vi "Array Panel Async.vi"(8 "ExecAnchor":refnum<class "ExecAnchor.lvclass">, 10 "Container":refnum<vi>, 11 "PanelArray in":refnum<class "ArrayManager.lvclass">) -> ()   [LabVIEW 2020, in "OOPanel.lvlib" / "ArrayManager.lvclass"]
uses:
  ArrayManager.lvclass
  lv-exec-anchor/ExecAnchor/ExecAnchor.lvclass
  UI State.ctl
  Events.ctl
  Scroll Into View.ctl
  ArrayManager.lvclass/ArrayManager.ctl
  ArrayPanel/ArrayPanel.lvclass
  C:/dev/lv20CE/relink/lv-oopanel/OOPanel/Panel/Panel.lvclass
  Panel/Panel.lvclass
panel:
  out "Page Size":dbl
  in  "Scrollbar":i32(c297)
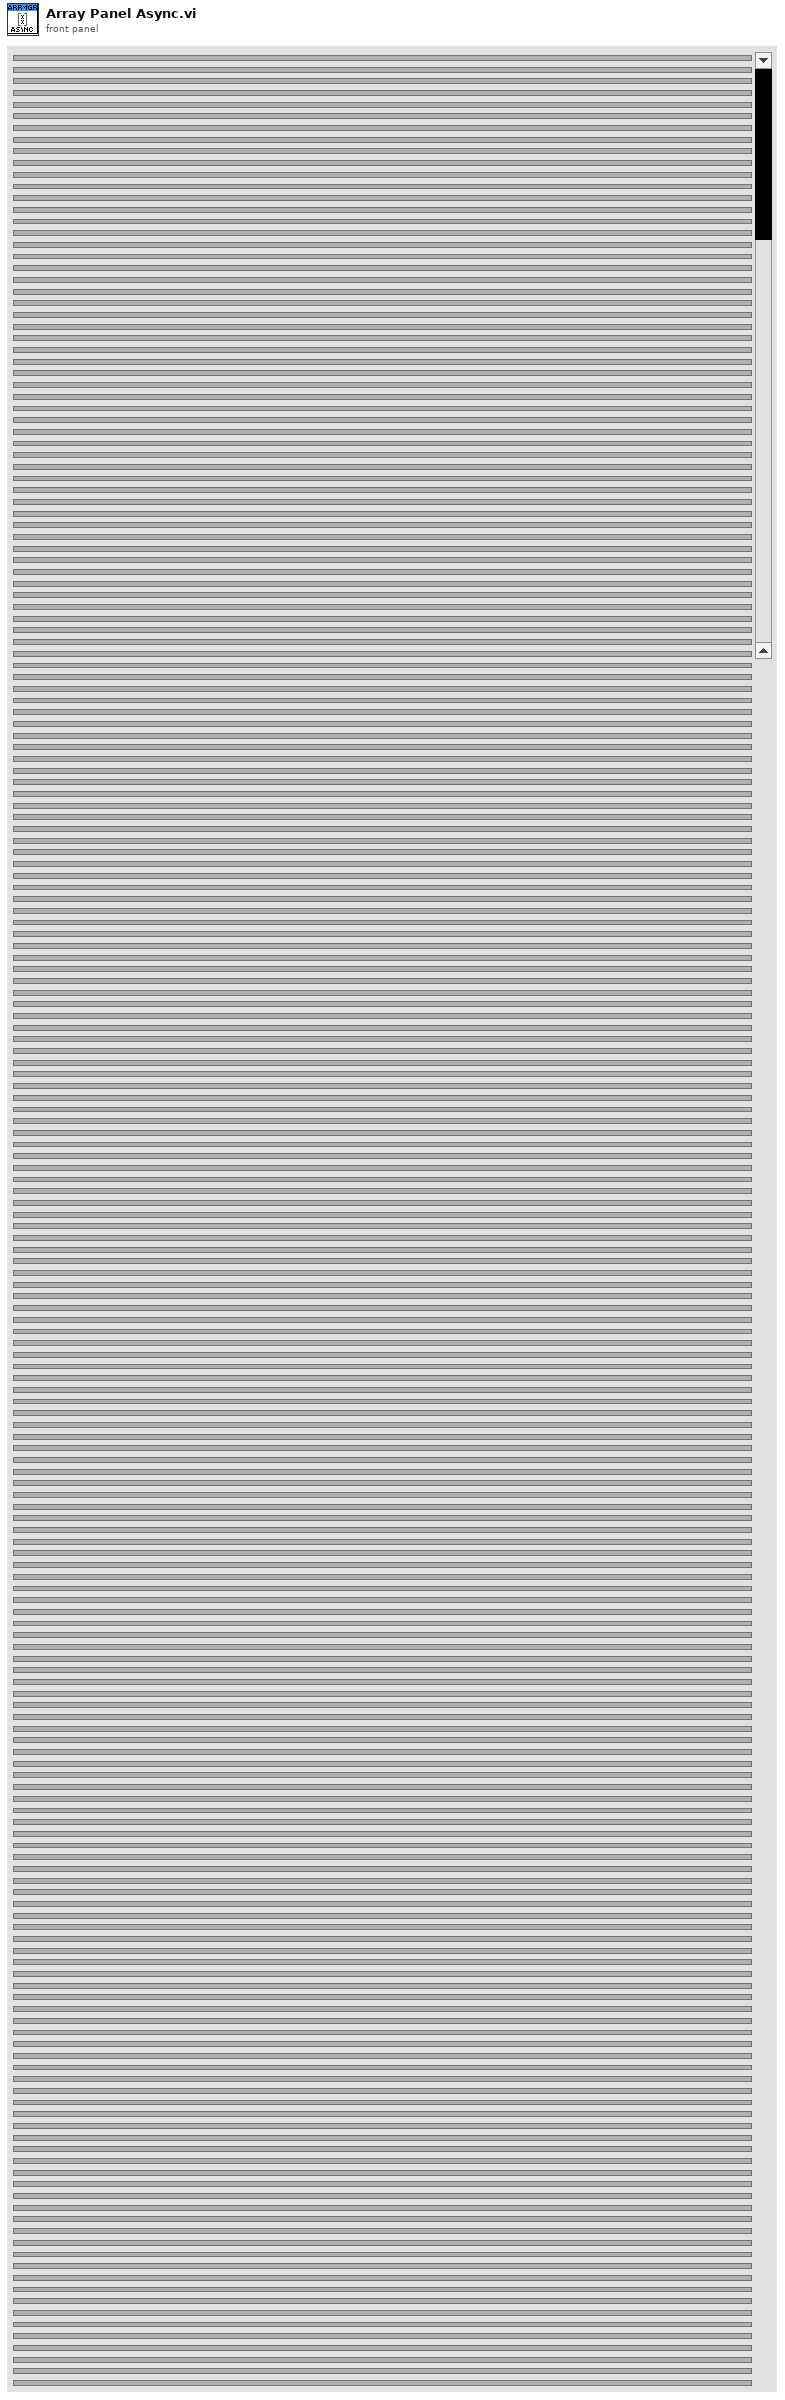
[diagram p1: front panel]
types:
  T1 = typedef "OOPanel.lvlib/ArrayManager.lvclass/UI State.ctl" = enum16{"Init", "Run", "Close"}
  T2 = cluster{"Panel":refnum<event-registration>, "ExecAnchor":refnum<event-registration>}
  T3 = typedef "OOPanel.lvlib/ArrayManager.lvclass/State Ref.ctl" = cluster{"Running":bool, "Borders":bool, "Total Height":dbl, "Scroll Visible":bool, "Background":u32}
  T4 = typedef "OOPanel.lvlib/ArrayManager.lvclass/UI Refs.ctl" = cluster{"SubPanels":refnum<vi>[], "Scrollbar":refnum<vi>, "Panel VI":refnum<vi>, "Container":refnum<vi>}
  T5 = typedef "OOPanel.lvlib/ArrayManager.lvclass/Events.ctl" = cluster{"Stop":refnum<user-event>, "Update":refnum<user-event>, "Scroll":refnum<user-event>, "Set BG":refnum<user-event>, "Scroll To Panel":refnum<user-event>, "Highlight":refnum<user-event>}
  T6 = typedef "OOPanel.lvlib/Desired Size.ctl" = cluster{"Width":u32, "Height":u32}
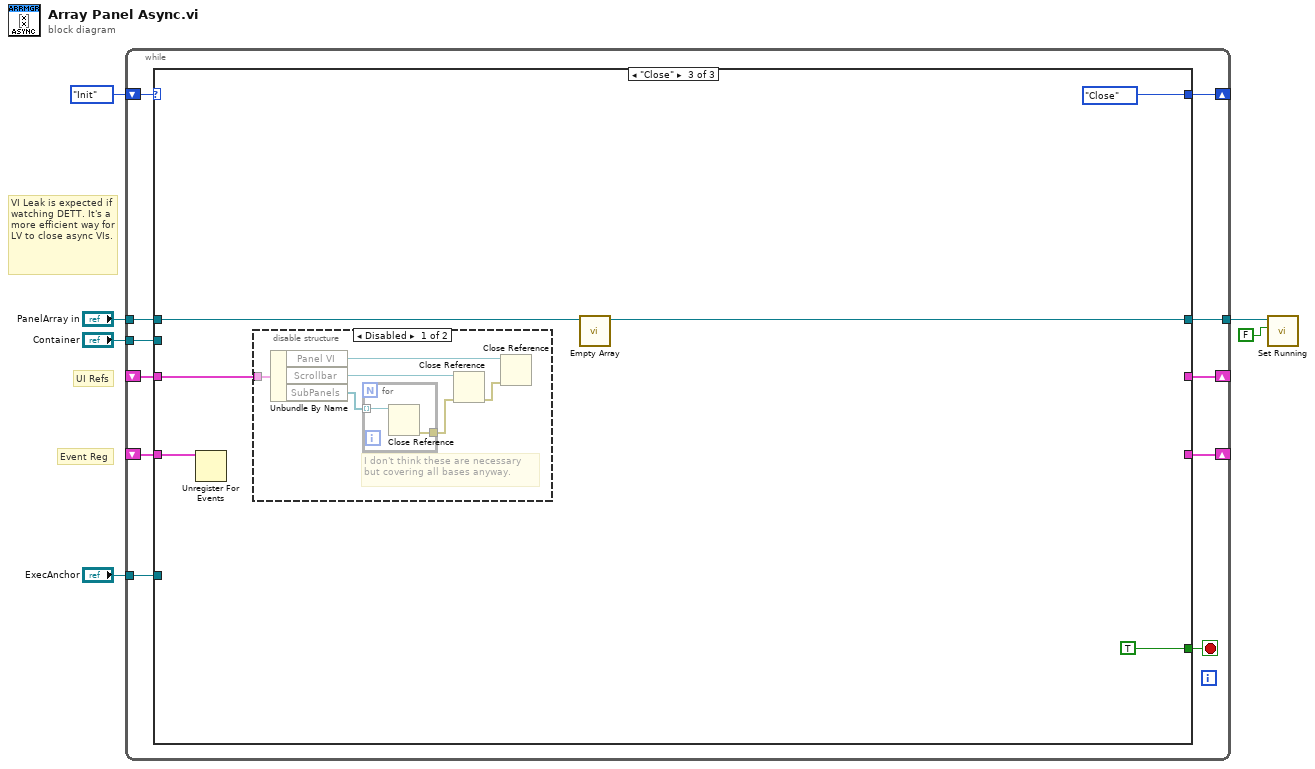
[diagram p0: block diagram]
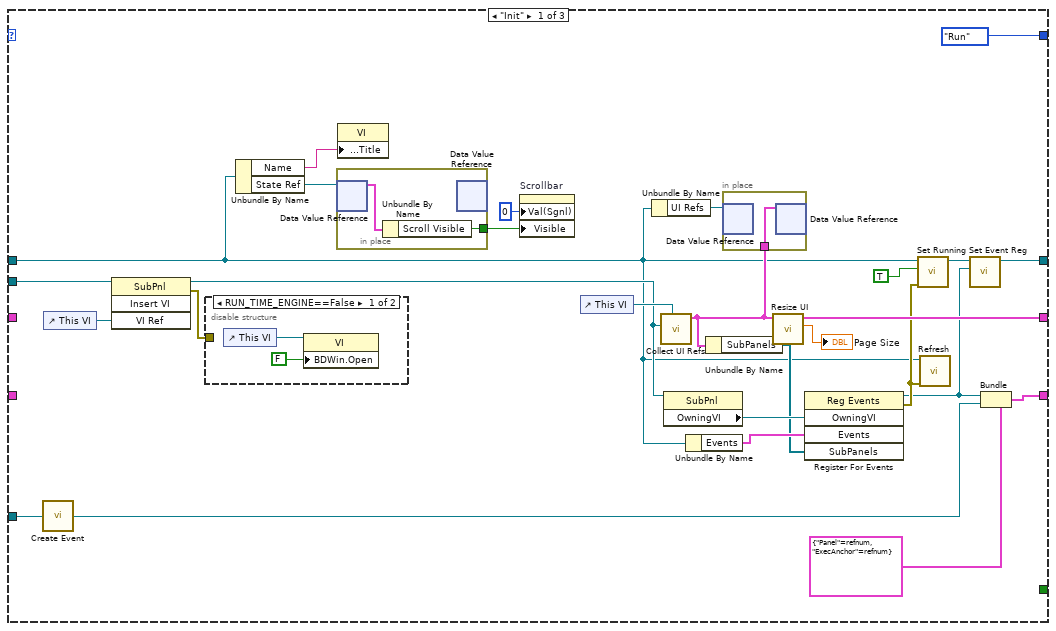
[diagram p2: hidden frame]
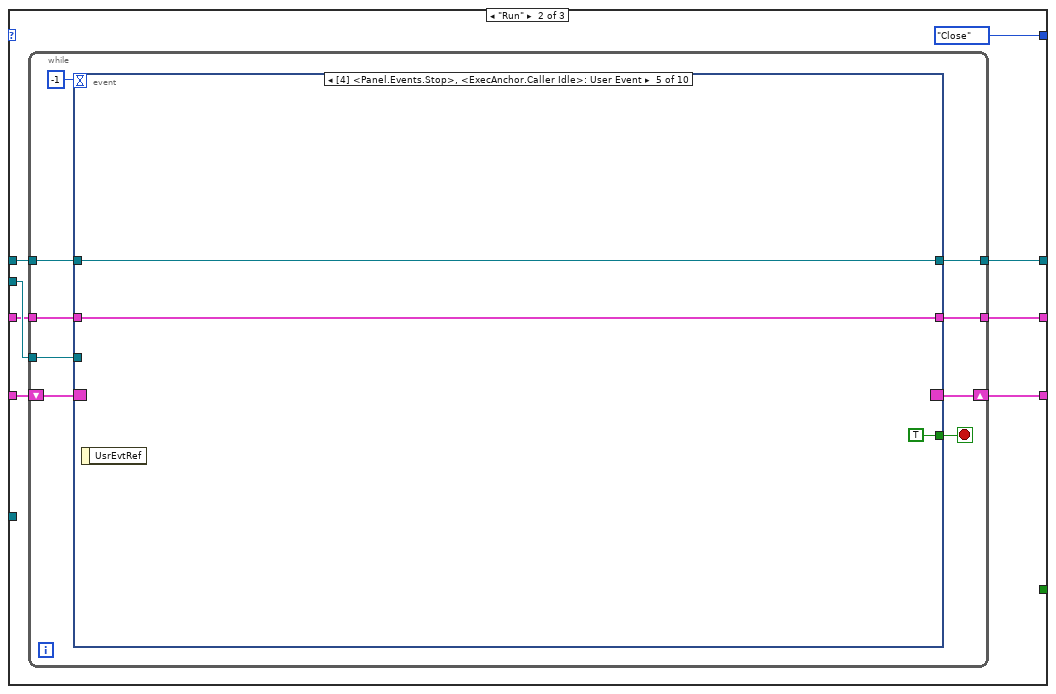
[diagram p4: hidden frame]
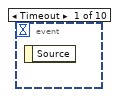
[diagram p5: hidden frame]
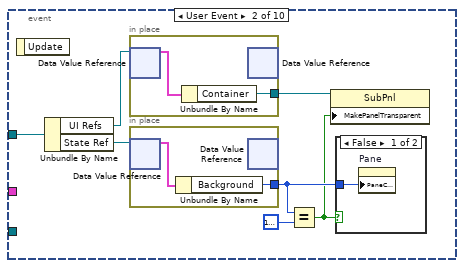
[diagram p6: hidden frame]
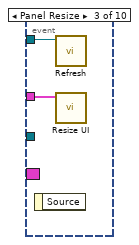
[diagram p8: hidden frame]
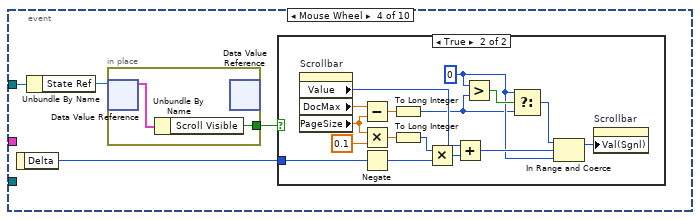
[diagram p9: hidden frame]
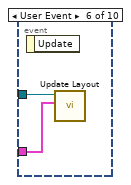
[diagram p11: hidden frame]
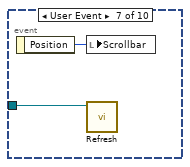
[diagram p12: hidden frame]
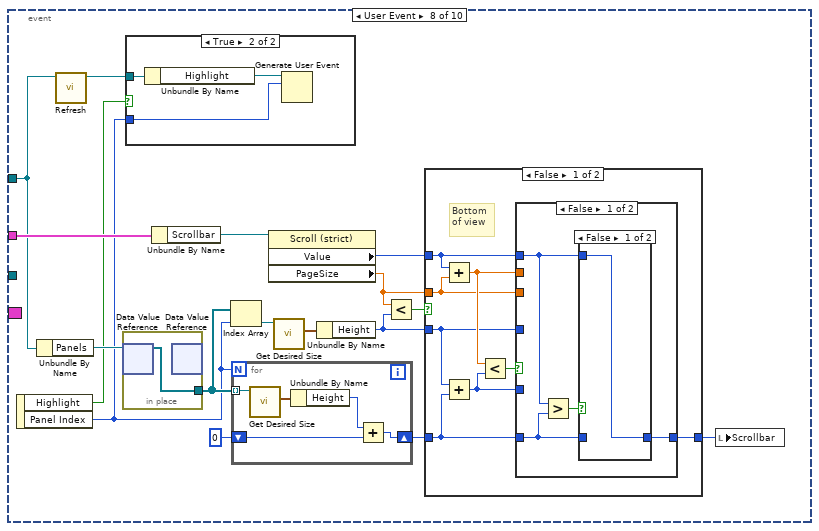
[diagram p13: hidden frame]
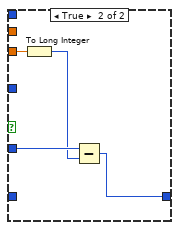
[diagram p16: hidden frame]
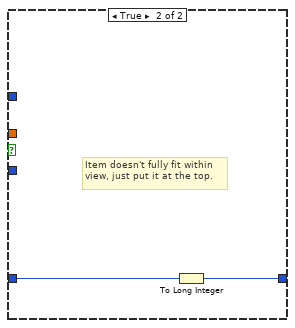
[diagram p17: hidden frame]
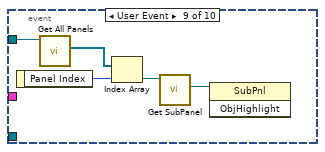
[diagram p18: hidden frame]
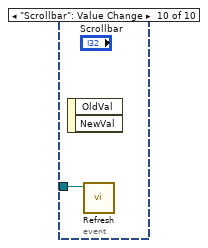
[diagram p19: hidden frame]
diagram:
  # "VI Leak is expected if watching DETT. It's a more efficient way for LV to close async VIs."
  # "Event Reg"
  # "UI Refs"
  n1 = while {
    shift-right: [w16] -> _
    shift-left: UI_State."Init" ("UI State") -> [w17]
    tunnel: "PanelArray in" -> [w15]
    tunnel: "Container" -> [w13]
    shift-right: [w12] -> _
    shift-left: _ -> [w11]
    shift-right: [w10] -> _
    shift-left: _ -> [w9]
    tunnel: [w8] -> w4
    tunnel: "ExecAnchor" -> [w7]
    stop <- w14 stop-if-true
    n2 = case shown="\"Close\"" w17 {
      tunnel: [UI_State."Run" ("UI State") UI_State."Close" ("UI State") UI_State."Close" ("UI State")] -> w16
      tunnel: w15 -> [w22 w56 w163]
      tunnel: [_ _ TRUE] -> w14
      tunnel: w13 -> [w37 w55 _]
      tunnel: [w18 w54 _] -> w12
      tunnel: w11 -> [_ w53 w165]
      tunnel: [w40 w51 _] -> w10
      tunnel: w9 -> [_ w52 w164]
      tunnel: [w25 w50 w162] -> w8
      tunnel: w7 -> [w21 _ _]
      frame "Init" {
        n3 = call "Create Event.vi"("ExecAnchor in"=w21) -> ("Event Reg"=w20:refnum<event-registration>)  [unwired: 3 in, 1 out]
        n4 = control-ref of="This VI"() -> (w36:refnum<vi>)
        n5 = invoke class="SubPnl" method="Insert VI"(reference=w37, "VI Ref"=w36) -> (reference out=w35:refnum<vi>, error out=w34:errorcluster)  [unwired: 2 in, 2 out]
        n6 = disable-structure shown="RUN_TIME_ENGINE==False" {
          disable-tunnel: w34 -> [_ _]
          frame condition #0 (active) {
            n7 = control-ref of="This VI"() -> (w49:refnum<vi>)
            n8 = property class="VI"(reference=w49, "BDWin.Open"=FALSE ("Block Diagram Window:Open")) -> ()  [unwired: 1 in, 2 out]
          }
          frame condition #1 {
          }
        }
        n9 = Unbundle By Name(w22) -> ("Name"=w23:string, "State Ref"=w31:refnum<data-value>)
        n10 = in-place {
          in-place-border: [w46] -> w30
          n11 = in-place-dvr #1(w31) -> (w47:T3)  [unwired: 1 out]
          n12 = Unbundle By Name(w47) -> ("Scroll Visible"=w46:bool)
          n13 = in-place-dvr #1() -> ()  [unwired: 1 in, 2 out]
        }
        n14 = property class="VI"("Front Panel.Title"=w23) -> ()  [unwired: 2 in, 2 out]
        n15 = property on="Scrollbar" class="Scroll (strict)"("Val(Sgnl)"=0 ("Value (Signaling)"), "Visible"=w30) -> ()  [unwired: 2 in, 2 out]
        n16 = control-ref of="This VI"() -> (w43:refnum<vi>)
        n17 = Unbundle By Name(w22) -> ("UI Refs"=w29:refnum<data-value>)
        n18 = call "Collect UI Refs.vi"("VI Refnum"=w43, "Container"=w35) -> ("UI Refs"=w28:T4)  [unwired: 9 in]
        n19 = property class="SubPnl"(reference=w35) -> ("OwningVI"=w41:refnum<vi>)  [unwired: 1 in, 2 out]
        n20 = Unbundle By Name(w22) -> ("Events"=w39:T5)
        n21 = Unbundle By Name(w28) -> ("SubPanels"=w32:refnum<vi>[])
        n22 = in-place {
          in-place-border: w28 -> [w45]
          n23 = in-place-dvr #2(w29) -> ()  [unwired: 2 out]
          n24 = in-place-dvr #2(w45) -> ()  [unwired: 2 out]
        }
        n25 = call "Resize UI.vi"("UI Refs In"=w28) -> ("Page Size"=→"Page Size":dbl, "UI Refs"=w40:T4)  [unwired: 9 in]
        n26 = register-events(w41, w39, w32) -> (reference out=w24:refnum<event-registration>, error out=w27:errorcluster)  [unwired: 2 in]
        n27 = call "Set Running.vi"("error in (no error)"=w27, "Running"=TRUE, "ArrayManager in"=w22) -> ("ArrayManager out"=w26:refnum<class "ArrayManager.lvclass">)  [unwired: 7 in, 1 out]
        n28 = call "Refresh.vi"("error in (no error)"=w27, "ArrayManager in"=w22) -> ()  [unwired: 8 in, 2 out]
        n29 = call "Set Event Reg.vi"("Event Reg"=w24, "ArrayManager in"=w26) -> ("ArrayManager out"=w25:refnum<class "ArrayManager.lvclass">)  [unwired: 8 in, 1 out]
        n30 = Bundle(cluster=T2 {"Panel"=refnum, "ExecAnchor"=refnum}, "Panel"=w24, "ExecAnchor"=w20) -> (w18:T2)
      }
      frame "Run" {
        n31 = while {
          tunnel: w56 -> [w65]
          tunnel: w55 -> [w64]
          shift-right: [w63] -> w54
          shift-left: w53 -> [w62]
          tunnel: w52 -> [w61]
          tunnel: [w60] -> w51
          tunnel: [w58] -> w50
          stop <- w59 stop-if-true
          n32 = event shown="[4] <Panel.Events.Stop>, <ExecAnchor.Caller Idle>: User Event" {
            selector: w62 -> [_ _ _ _ _ _ _ _ _ _]
            dyn-events: [_ _ _ _ _ _ _ _ _ _] -> w63
            timeout: -1 -> [_ _ _ _ _ _ _ _ _ _]
            tunnel: w65 -> [_ w72 w79 w82 w103 w107 w108 w117 w160 w161]
            tunnel: w64 -> [_ _ _ _ _ _ _ _ _ _]
            tunnel: w61 -> [_ _ w80 _ w105 w106 _ w121 _ _]
            tunnel: [_ _ _ _ w105 _ _ _ _ _] -> w60
            tunnel: [_ _ _ _ TRUE _ _ _ _ _] -> w59
            tunnel: [_ _ _ _ w103 _ _ _ _ _] -> w58
            event Timeout {
              n33 = event-data() -> ()  [unwired: 1 in, 1 out]
            }
            event User Event {
              n34 = event-data() -> ()  [unwired: 1 in, 1 out]
              n35 = Unbundle By Name(w72) -> ("UI Refs"=w69:refnum<data-value>, "State Ref"=w73:refnum<data-value>)
              n36 = in-place {
                in-place-border: [w74] -> w68
                n37 = in-place-dvr #3(w69) -> (w75:T4)  [unwired: 1 out]
                n38 = Unbundle By Name(w75) -> ("Container"=w74:refnum<vi>)
                n39 = in-place-dvr #3() -> ()  [unwired: 1 in, 2 out]
              }
              n40 = in-place {
                in-place-border: [w77] -> w70
                n41 = in-place-dvr #4(w73) -> (w78:T3)  [unwired: 1 out]
                n42 = Unbundle By Name(w78) -> ("Background"=w77:u32)
                n43 = in-place-dvr #4() -> ()  [unwired: 1 in, 2 out]
              }
              n44 = Equal?(x=w70, y=u32 16777216) -> (x = y?=w67:bool)
              n45 = property class="SubPnl"(reference=w68, "MakePanelTransparent"=w67) -> ()  [unwired: 1 in, 2 out]
              n46 = case shown="False" w67 {
                tunnel: w70 -> [w76 _]
                frame False {
                  n47 = property on="Pane" class="Pane"("PaneColor"=w76) -> ()  [unwired: 2 in, 2 out]
                }
                frame True {
                }
              }
            }
            event Panel Resize {
              n48 = event-data() -> ()  [unwired: 1 in, 1 out]
              n49 = call "Refresh.vi"("ArrayManager in"=w79) -> ()  [unwired: 9 in, 2 out]
              n50 = call "Resize UI.vi"("UI Refs In"=w80) -> ()  [unwired: 9 in, 2 out]
            }
            event Mouse Wheel {
              n51 = event-data() -> ("Delta"=w84:i32)  [unwired: 1 in]
              n52 = Unbundle By Name(w82) -> ("State Ref"=w83:refnum<data-value>)
              n53 = in-place {
                in-place-border: [w85] -> w81
                n54 = in-place-dvr #5(w83) -> (w86:T3)  [unwired: 1 out]
                n55 = Unbundle By Name(w86) -> ("Scroll Visible"=w85:bool)
                n56 = in-place-dvr #5() -> ()  [unwired: 1 in, 2 out]
              }
              n57 = case shown="True" w81 {
                tunnel: w84 -> [_ w87]
                frame False {
                }
                frame True {
                  w90 = 0 ("lower limit")
                  n58 = property on="Scrollbar" class="Scroll (strict)"() -> ("Value"=w98:i32, "DocMax"=w96:dbl, "PageSize"=w95:dbl)  [unwired: 2 in, 2 out]
                  n59 = Subtract(x=w96, y=w95) -> (x-y=w94:dbl)
                  n60 = Multiply(x=w95, y=0.1) -> (x*y=w101:dbl)
                  n61 = Negate(x=w87) -> (-x=w92:i32)
                  n62 = To Long Integer(number=w94) -> (32bit integer=w89:i32)
                  n63 = To Long Integer(number=w101) -> (32bit integer=w99:i32)
                  n64 = Multiply(x=w99, y=w92) -> (x*y=w100:i32)
                  n65 = Add(x=w98, y=w100) -> (x+y=w97:i32)
                  n66 = Greater?(x=w90, y=w89) -> (0:w91:bool)
                  n67 = Select(t=w90, s=w91, f=w89) -> (s? t:f=w88:i32)
                  n68 = In Range and Coerce(upper limit=w88, x=w97, lower limit=w90) -> (coerced(x)=w93:i32)  [unwired: 1 out]
                  n69 = property on="Scrollbar" class="Scroll (strict)"("Val(Sgnl)"=w93) -> ()  [unwired: 2 in, 2 out]
                }
              }
            }
            event User Event {
              n70 = event-data() -> ()  [unwired: 1 in, 1 out]
            }
            event User Event {
              n71 = event-data() -> ()  [unwired: 1 in, 1 out]
              n72 = call "Update Layout.vi"("UI Refs"=w106, "ArrayManager in"=w107) -> ()  [unwired: 8 in, 2 out]
            }
            event User Event {
              n73 = event-data() -> ("Position"=w109:i32)  [unwired: 1 in]
              n74 = local write "Scrollbar"(w109) -> ()
              n75 = call "Refresh.vi"("ArrayManager in"=w108) -> ()  [unwired: 9 in, 2 out]
            }
            event User Event {
              n76 = event-data() -> ("Highlight"=w112:bool, "Panel Index"=w110:i32)  [unwired: 1 in]
              n77 = Unbundle By Name(w117) -> ("Panels"=w126:refnum<data-value>)
              n78 = call "Refresh.vi"("ArrayManager in"=w117) -> ("ArrayManager out"=w111:refnum<class "ArrayManager.lvclass">)  [unwired: 9 in, 1 out]
              n79 = in-place {
                in-place-border: [w155] -> w124
                n80 = in-place-dvr #6(w126) -> (w155:refnum<class "ArrayPanel.lvclass">[])  [unwired: 1 out]
                n81 = in-place-dvr #6() -> ()  [unwired: 1 in, 2 out]
              }
              n82 = case shown="True" w112 {
                tunnel: w111 -> [_ w129]
                tunnel: w110 -> [_ w127]
                frame False {
                }
                frame True {
                  n83 = Unbundle By Name(w129) -> ("Highlight"=w128:refnum<user-event>)
                  n84 = Generate User Event(user event=w128, event data cluster=w127) -> ()  [unwired: 2 in, 2 out]
                }
              }
              n85 = Unbundle By Name(w121) -> ("Scrollbar"=w120:refnum<vi>)
              n86 = Index Array(array=w124, index=w110) -> (element=w123:refnum<class "ArrayPanel.lvclass">)
              n87 = for {
                N: w110 -> [_]
                tunnel: w124 -> [w154] mode=indexing
                shift-right: [w151] -> w118
                shift-left: u32 0 ("Height") -> [w152]
                n88 = call-dynamic "Get Desired Size.vi"("ArrayPanel in"=w154) -> ("Desired Size"=w153:T6)  [unwired: 8 in, 2 out]
                n89 = Unbundle By Name(w153) -> ("Height"=w150:u32)
                n90 = Add(x=w150, y=w152) -> (x+y=w151:u32)
              }
              n91 = property class="Scroll (strict)"(reference=w120) -> ("Value"=w113:i32, "PageSize"=w114:dbl)  [unwired: 1 in, 2 out]
              n92 = call-dynamic "Get Desired Size.vi"("ArrayPanel in"=w123) -> ("Desired Size"=w122:T6)  [unwired: 8 in, 2 out]
              n93 = Unbundle By Name(w122) -> ("Height"=w115:u32)
              n94 = Less?(x=w114, y=w115) -> (x < y?=w119:bool)
              n95 = case shown="False" w119 {
                tunnel: w118 -> [w136 w149]
                tunnel: [w134 w148] -> w116
                tunnel: w115 -> [w132 _]
                tunnel: w114 -> [w130 _]
                tunnel: w113 -> [w133 _]
                frame False {
                  # "Bottom of view"
                  n96 = Add(x=w133, y=w130) -> (x+y=w135:dbl)
                  n97 = Add(x=w132, y=w136) -> (x+y=w131:u32)
                  n98 = Less?(x=w135, y=w131) -> (x < y?=w137:bool)
                  n99 = case shown="False" w137 {
                    tunnel: w136 -> [w138 _]
                    tunnel: w135 -> [_ _]
                    tunnel: [w139 w145] -> w134
                    tunnel: w133 -> [w140 _]
                    tunnel: w132 -> [_ _]
                    tunnel: w131 -> [_ w147]
                    tunnel: w130 -> [_ w146]
                    frame False {
                      n100 = Greater?(x=w140, y=w138) -> (0:w141:bool)
                      n101 = case shown="False" w141 {
                        tunnel: w140 -> [w142 _]
                        tunnel: [w142 w143] -> w139
                        tunnel: w138 -> [_ w143]
                        frame False {
                        }
                        frame True {
                        }
                      }
                    }
                    frame True {
                      n102 = To Long Integer(number=w146) -> (32bit integer=w144:i32)
                      n103 = Subtract(x=w147, y=w144) -> (x-y=w145:u32)
                    }
                  }
                }
                frame True {
                  # "Item doesn't fully fit within view, just put it at the top."
                  n104 = To Long Integer(number=w149) -> (32bit integer=w148:i32)
                }
              }
              n105 = local write "Scrollbar"(w116) -> ()
            }
            event User Event {
              n106 = event-data() -> ("Panel Index"=w158:i32)  [unwired: 1 in]
              n107 = call "Get All Panels.vi"("PanelArray in"=w160) -> ("Panels"=w159:refnum<class "ArrayPanel.lvclass">[])  [unwired: 8 in, 2 out]
              n108 = Index Array(array=w159, index=w158) -> (element=w157:refnum<class "ArrayPanel.lvclass">)
              n109 = call "Get SubPanel.vi"("Panel in"=w157) -> ("SubPanel"=w156:refnum<vi>)  [unwired: 8 in, 2 out]
              n110 = invoke class="SubPnl" method="ObjHighlight"(reference=w156) -> ()  [unwired: 2 in, 3 out]
            }
            event "Scrollbar": Value Change {
              n111 = event-data() -> ()  [unwired: 1 in, 2 out]
              n112 = call "Refresh.vi"("ArrayManager in"=w161) -> ()  [unwired: 9 in, 2 out]
            }
          }
        }
      }
      frame "Close" {
        n113 = Unregister For Events(event registration refnum=w165) -> ()  [unwired: 1 in, 1 out]
        n114 = disable-structure shown="Disabled" {
          disable-tunnel: w164 -> [w173 _]
          frame Disabled {
            # "I don't think these are necessary but covering all bases anyway."
            n115 = Unbundle By Name(w173) -> ("Panel VI"=w171:refnum<vi>, "Scrollbar"=w172:refnum<vi>, "SubPanels"=w169:refnum<vi>[])
            n116 = for {
              tunnel: w169 -> [w175] mode=indexing
              tunnel: [w174] -> w168
              n117 = Close Reference(reference=w175) -> (error out=w174:errorcluster)  [unwired: 1 in]
            }
            n118 = Close Reference(reference=w172, error in (no error)=w168) -> (error out=w170:errorcluster)
            n119 = Close Reference(reference=w171, error in (no error)=w170) -> ()  [unwired: 1 out]
          }
          frame Enabled {
          }
        }
        n120 = call "Empty Array.vi"("ArrayManager in"=w163) -> ("ArrayManager out"=w162:refnum<class "ArrayManager.lvclass">)  [unwired: 9 in, 1 out]
      }
    }
  }
  n121 = call "Set Running.vi"("Running"=FALSE, "ArrayManager in"=w4) -> ()  [unwired: 8 in, 2 out]
